vi "VIH ProjFile - Control Rules Array - Write.vi"(8 "error in":errorcluster, 9 "Control Rules":T1[](array[typedef]), 10 "Property Name":string, 11 "XML Parent Item":refnum<k20>) -> (0 "error out":errorcluster, 3 "dup XML Parent Item":refnum<k20>)   [LabVIEW 2014]
doc: "::: VI Helpeks :::\nCopyright (c) 2000-2026 Konstantin Shifershteyn. All rights reserved."
uses:
  _VIH HelpGen.llb/VIH HelpGen Typedef - Cluster - Control Rule.ctl
  _VIH HelpGen.llb/VIH HelpGen Typedef - Enum - Description Mode.ctl
  _VIH HelpGen.llb/VIH HelpGen Typedef - Enum - Default,Enable,Disable.ctl
  _VIH HelpGen.llb/VIH HelpGen Typedef - Cluster - Enum Value Info.ctl
  <vilib>/xml/Close Reference(Node).vi
  <resource>/objmgr/DOMUserDefRef.rc
  <vilib>/xml/NI_XML.lvlib
panel:
  in  "Control Rule (data)":T1
  # "VI Helpeks\nCopyright (c) 2012-2026 Konstantin Shifershteyn"
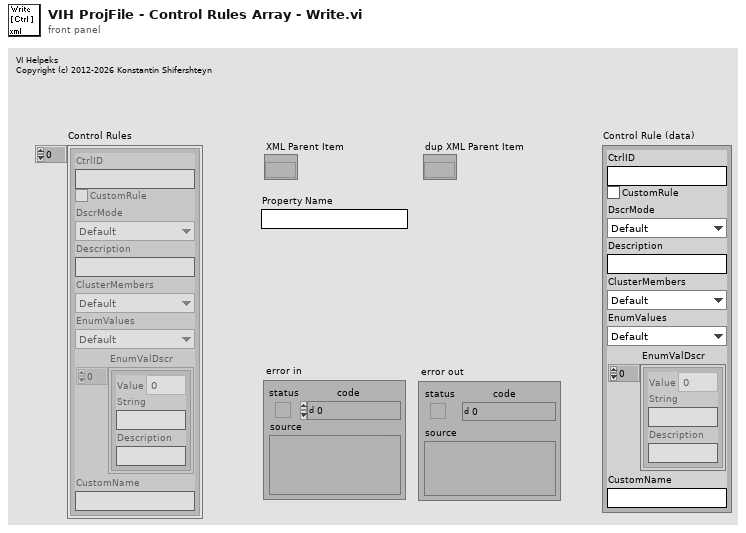
[diagram p1: front panel]
types:
  T1 = typedef "VIH HelpGen Typedef - Cluster - Control Rule.ctl" = cluster{"CtrlID":string, "CustomRule":bool, "DscrMode":T2, "Description":string, "ClusterMembers":T3, "EnumValues":T3, "EnumValDscr":T4[], "CustomName":string}
  T2 = typedef "VIH HelpGen Typedef - Enum - Description Mode.ctl" = enum16{"Default", "Description", "Description1", "Description2", "Custom", "None"}
  T3 = typedef "VIH HelpGen Typedef - Enum - Default,Enable,Disable.ctl" = enum16{"Default", "Enable", "Disable"}
  T4 = typedef "VIH HelpGen Typedef - Cluster - Enum Value Info.ctl" = cluster{"Value":ext, "String":string, "Description":string}
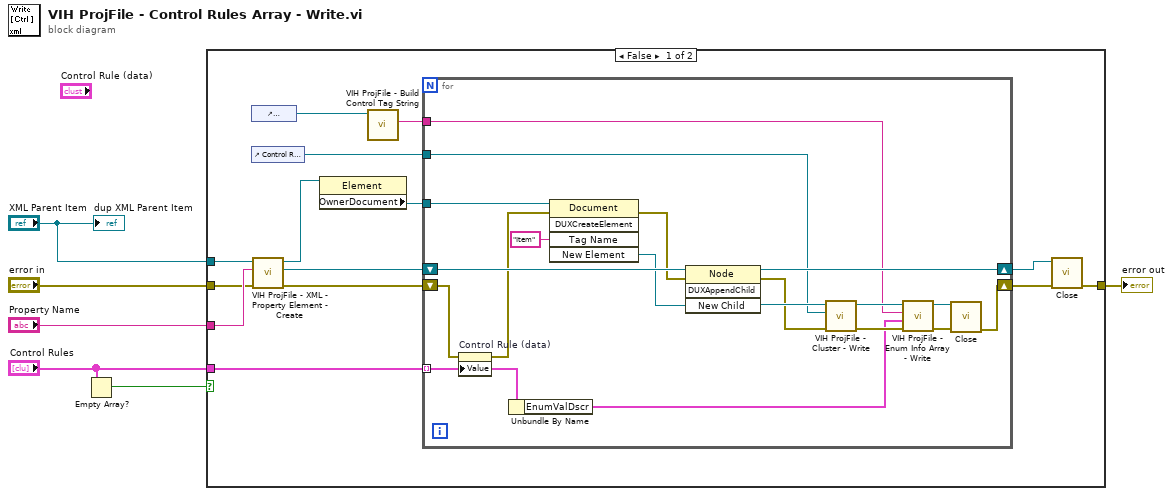
[diagram p0: block diagram]
diagram:
  n1 = Empty Array?(array="Control Rules") -> (empty?=w1:bool)
  n2 = case shown="False" w1 {
    tunnel: [w10 w39] -> w6
    tunnel: "XML Parent Item" -> [w13 _]
    tunnel: "Property Name" -> [w18 _]
    tunnel: "Control Rules" -> [w19 _]
    tunnel: "error in" -> [w12 w39]
    frame False {
      n3 = control-ref of="EnumValDscr"() -> (w8:refnum<vi>)
      n4 = control-ref of="Control Rule (data)"() -> (w9:refnum<vi>)
      n5 = call "VIH ProjFile - XML - Property Element - Create.vi"("error in"=w12, "Property Name"=w18, "XML Parent Item"=w13) -> ("error out"=w16:errorcluster, "New Child"=w17:refnum<k20>, "dup XML Parent Item"=w14:refnum<k20>)  [unwired: 6 in]
      n6 = property class="Element"(reference=w14) -> ("OwnerDocument"=w15:refnum<k20>)  [unwired: 1 in, 2 out]
      n7 = call "VIH ProjFile - Build Control Tag String.vi"("Ctl Refnum"=w8) -> ("Control Tag"=w7:string)  [unwired: 6 in, 4 out]
      n8 = for {
        shift-right: [w31] -> w11
        shift-left: w16 -> [w35]
        tunnel: w15 -> [w37]
        shift-right: [w32] -> w20
        shift-left: w17 -> [w36]
        tunnel: w19 -> [w24] mode=indexing
        tunnel: w9 -> [w22]
        tunnel: w7 -> [w21]
        n9 = property on="Control Rule (data)" class="Clust (strict)"(error in=w35, "Value"=w24) -> (error out=w34:errorcluster)  [unwired: 1 in, 1 out]
        n10 = Unbundle By Name(w24) -> ("EnumValDscr"=w23:T4[])
        n11 = invoke class="Document" method="DUXCreateElement"(reference=w37, error in=w34, "Tag Name"="Item") -> (error out=w33:errorcluster, "New Element"=w30:refnum<k20>)  [unwired: 2 in, 3 out]
        n12 = invoke class="Node" method="DUXAppendChild"(reference=w36, error in=w33, "New Child"=w30) -> (reference out=w32:refnum<k20>, error out=w28:errorcluster)  [unwired: 1 in, 2 out]
        n13 = call "VIH ProjFile - Cluster - Write.vi"("error in"=w28, "Ctl Refnum"=w22, "XML Parent Item"=w30) -> ("error out"=w27:errorcluster, "dup XML Parent Item"=w29:refnum<k20>)  [unwired: 7 in]
        n14 = call "VIH ProjFile - Enum Info Array - Write.vi"("error in"=w27, "EnumValDscr"=w23, "Property Name"=w21, "XML Parent Item"=w29) -> ("error out"=w26:errorcluster, "dup XML Parent Item"=w25:refnum<k20>)  [unwired: 6 in]
        n15 = call-poly <vilib>:"Close.vi"("error in (no error)"=w26, "node"=w25) -> ("error out"=w31:errorcluster)  [unwired: 7 in]
      }
      n16 = call-poly <vilib>:"Close.vi"("error in (no error)"=w11, "node"=w20) -> ("error out"=w10:errorcluster)  [unwired: 7 in]
    }
    frame True {
    }
  }
  "error out" <- w6
  "dup XML Parent Item" <- "XML Parent Item"
